vi "DCW_Limiter.vi"(0 "DCW HI SET current value(mA)":sgl=11.0 min=0.001 max=11 format="%.3f", 5 "DCW LO SET current value(mA)":sgl min=0 max=10.9 format="%.3f", 7 "DCW Test Time(S)":sgl=0.5 min=0.5 max=999.9 format="%.1f", 9 "Ramp Time":sgl=0.1 min=0.1 max=999.9 format="%.1f", 11 "DCW voltage(kV)":sgl=0.1 min=0.1 max=6.1 format="%.3f") -> (4 "DCW voltage(kV)":string, 6 "Ramp Time":string, 8 "DCW LO SET current value(mA)":string, 10 "DCW HI SET current value(mA)":string, 15 "DCW Test Time(S)":string)   [LabVIEW 2021]
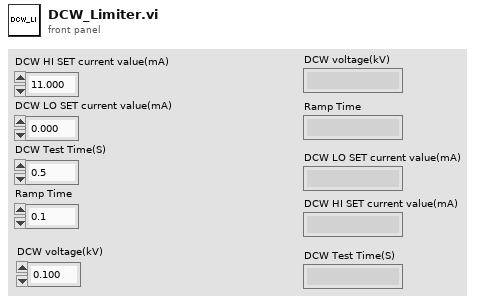
[diagram p1: front panel]
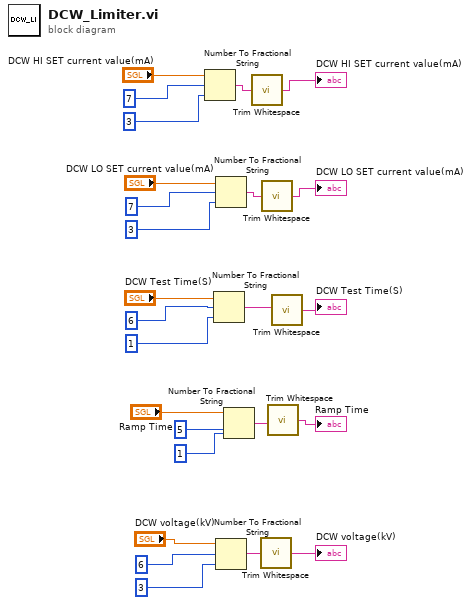
[diagram p0: block diagram]
diagram:
  n1 = Number To Fractional String(number="DCW HI SET current value(mA)", width (-)=i16 7, precision (6)=i16 3) -> (F-format string=w10:string)  [unwired: 1 in]
  n2 = Number To Fractional String(number="DCW Test Time(S)", width (-)=i16 6, precision (6)=i16 1 ("width (-)")) -> (F-format string=w6:string)  [unwired: 1 in]
  n3 = Number To Fractional String(number="DCW LO SET current value(mA)", width (-)=i16 7, precision (6)=i16 3) -> (F-format string=w8:string)  [unwired: 1 in]
  n4 = Number To Fractional String(number="DCW voltage(kV)", width (-)=i16 6, precision (6)=i16 3) -> (F-format string=w2:string)  [unwired: 1 in]
  n5 = Number To Fractional String(number="Ramp Time", width (-)=i16 5, precision (6)=i16 1) -> (F-format string=w4:string)  [unwired: 1 in]
  n6 = call <vilib>:"Trim Whitespace.vi"("string"=w10) -> ("trimmed string"=→"DCW HI SET current value(mA)":string)  [unwired: 1 in]
  n7 = call <vilib>:"Trim Whitespace.vi"("string"=w2) -> ("trimmed string"=→"DCW voltage(kV)":string)  [unwired: 1 in]
  n8 = call <vilib>:"Trim Whitespace.vi"("string"=w8) -> ("trimmed string"=→"DCW LO SET current value(mA)":string)  [unwired: 1 in]
  n9 = call <vilib>:"Trim Whitespace.vi"("string"=w4) -> ("trimmed string"=→"Ramp Time":string)  [unwired: 1 in]
  n10 = call <vilib>:"Trim Whitespace.vi"("string"=w6) -> ("trimmed string"=→"DCW Test Time(S)":string)  [unwired: 1 in]
